vi "Configure Task Sync.vi"(7 "VolatusAPI":refnum<class "VolatusAPI.lvclass">, 8 "error in (no error)":errorcluster, 11 "DAQmx Task In":refnum<k21>) -> (0 "error out":errorcluster, 3 "DAQmx Task":refnum<k21>)   [LabVIEW 2025, in "VolatusDAQ.lvlib"]
uses:
  VolatusDAQ.lvlib
  <resource>/objmgr/daqmx.rc
  Volatus/VolatusAPI/VolatusAPI.lvclass
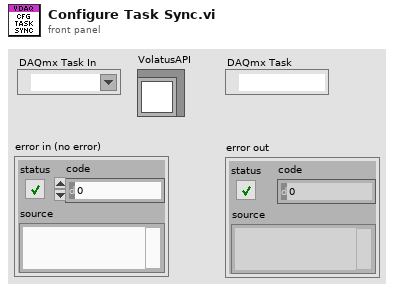
[diagram p1: front panel]
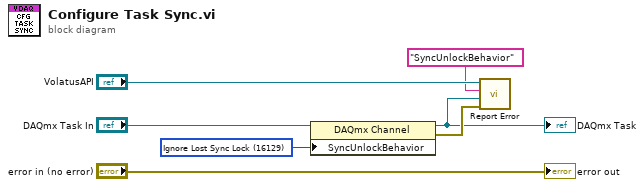
[diagram p0: block diagram]
diagram:
  w5 = 16129 items=["Stop Task and Error"=15862, "Ignore Lost Sync Lock"=16129] ("SyncUnlockBehavior")
  n1 = property class="DAQmx Channel"(reference="DAQmx Task In", "SyncUnlockBehavior"=w5) -> (reference out=w2:refnum<k21>, error out=w7:errorcluster)  [unwired: 1 in]
  "DAQmx Task" <- w2
  n2 = call "Report Error.vi"("error in (no error)"=w7, "Message"=w2, "Context"="SyncUnlockBehavior", "VolatusAPI in"="VolatusAPI") -> ()  [unwired: 6 in, 2 out]
  "error out" <- "error in (no error)"
